vi "RemoteVI Status.vi"() -> (4 "servers":T1(array[cluster]), 6 "text":string)   [LabVIEW 2020, in "RemoteVI.lvlib"]
doc: "The status of every RemoteVI share of this LabVIEW application instance (RemoteVI Start.vi, the Tools menu entry or RemoteVI Server), for your own UI or a log. Per share: port, url (the full link with its access token), target (the VI or window shared) and kind (VI or Window), whole network (FALSE: this computer only), running (the server loop updated it within the last 2 s), uptime s, the clients with their address, connected s and idle s (seconds since their last input, -1 when none yet), fps (frames made per second), kB per s sent, frames made, latency ms (last remote click or key to the next frame), view only and last error. text is the same as readable text (RemoteVI Status Text.vi). The server loops publish every 500 ms; this VI only reads, so it is cheap to call in a loop. RemoteVI Status Panel.vi shows it."
uses:
  RemoteVI.lvlib
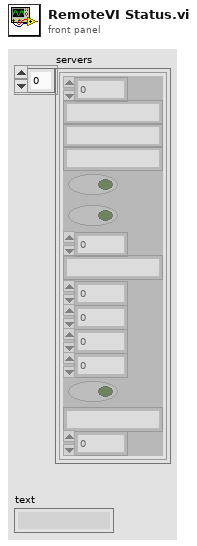
[diagram p1: front panel]
types:
  T1 = cluster{"port":u16, "url":string, "target":string, "kind":string, "whole network":bool, "running":bool, "uptime s":dbl, "clients":cluster{"address":string, "connected s":dbl, "idle s":dbl}[], "fps":dbl, "kB per s":dbl, "frames":u32, "latency ms":dbl, "view only":bool, "last error":string, "hWnd":u64}[]
  T2 = cluster{"port":u16, "url":string, "target":string, "kind":string, "whole network":bool, "started":dbl, "updated":dbl, "clients":cluster{"address":string, "since":dbl, "last input":dbl}[], "fps":dbl, "bytes per s":dbl, "frames":u32, "latency ms":dbl, "view only":bool, "last error":string, "hWnd":u64}[]
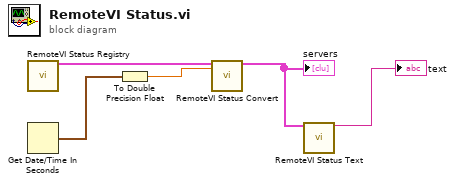
[diagram p0: block diagram]
diagram:
  n1 = call "RemoteVI Status Registry.vi"() -> ("servers"=w1:T2)  [unwired: 15 in]
  n2 = Get Date/Time In Seconds() -> (seconds since 1Jan1904=w2:timestamp)
  n3 = To Double Precision Float(number=w2) -> (double precision float=w3:dbl)
  n4 = call "RemoteVI Status Convert.vi"("raw"=w1, "now"=w3) -> ("status"=w4:T1)  [unwired: 13 in]
  "servers" <- w4
  n5 = call "RemoteVI Status Text.vi"("status"=w4) -> ("text"=→"text":string)  [unwired: 14 in]
